vi "MoveMouseCursor.vi"(0 "Left Position":i32, 5 "Right Position":i32, 11 "Error In":errorcluster) -> (15 "Error Out":errorcluster)   [LabVIEW 2019, in "Drona.lvlib"]
doc: "This VI moves mouse cursor to the given position"
uses:
  Drona.lvlib
  user32.dll
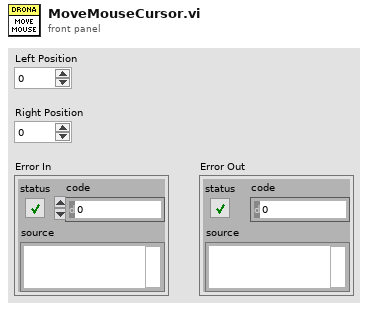
[diagram p1: front panel]
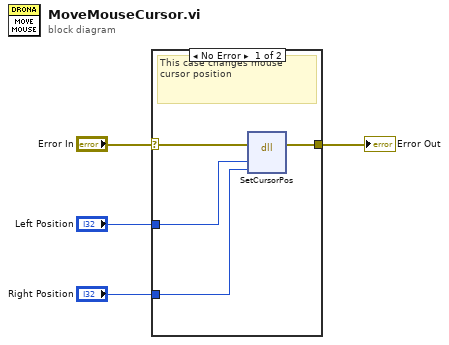
[diagram p0: block diagram]
diagram:
  n1 = case shown="No Error" "Error In" {
    selector: "Error In" -> [w5 w9]
    tunnel: [w8 w9] -> w4
    tunnel: "Right Position" -> [w7 _]
    tunnel: "Left Position" -> [w6 _]
    frame No Error {
      # "This case changes mouse cursor position"
      n2 = dll-call lib="user32.dll" fn="SetCursorPos"(error in=w5, "dx"=w6, "dy"=w7) -> (error out=w8:errorcluster)  [unwired: 5 in, 1 out]
    }
    frame Error {
      # "If error, this case pass that error message only"
    }
  }
  "Error Out" <- w4
